vi "test malformed json.vi"(8 "error in (no error)":errorcluster) -> (0 "error out":errorcluster, 3 "body":string)   [LabVIEW 2020, in "MCP Server tests.lvlib"]
doc: "A body that is not valid JSON cannot be read: JSON-RPC error -32700 (Parse error) with id null, even if the text contains something that looks like an id."
uses:
  MCP Server tests.lvlib
  <vilib>/JDP Science/JSONtext/Next JSON Value.vi
  <vilib>/JDP Science/JSONtext/String Subset.vi
  <vilib>/JDP Science/JSONtext/Parsing/Advance past next JSON Value (inlined COPY).vi
  <vilib>/JDP Science/JSONtext/Parsing/Advance past whitespace.vi
  <vilib>/JDP Science/JSONtext/Parsing/Advance past String.vi
  <vilib>/JDP Science/JSONtext/Parsing/Advance past Number.vi
  <vilib>/JDP Science/JSONtext/Parsing/Advance past Line Ending.vi
  <vilib>/JDP Science/JSONtext/Parsing/Parse Full Path or Item Name.vi
  <vilib>/JDP Science/JSONtext/Parsing/Advance past Array.vi
  <vilib>/JDP Science/JSONtext/Parsing/Advance past Object.vi
  <vilib>/JDP Science/JSONtext/support/Error Cluster From Code.vi
  <vilib>/JDP Science/JSONtext/Offset/Find Item Locations by Path.vi
  <vilib>/addons/_JKI Toolkits/Caraya/classes/Test/Test.lvclass
  <vilib>/JDP Science/JSONtext/JSONtext.lvlib
  <vilib>/addons/_JKI Toolkits/Caraya/classes/Assert/Assert.lvclass
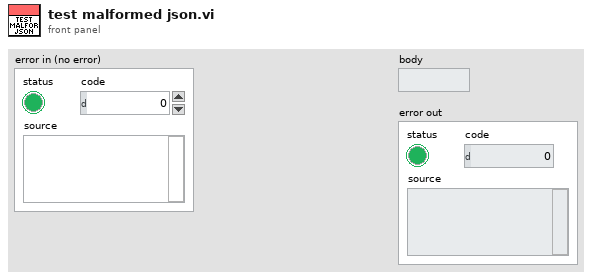
[diagram p1: front panel]
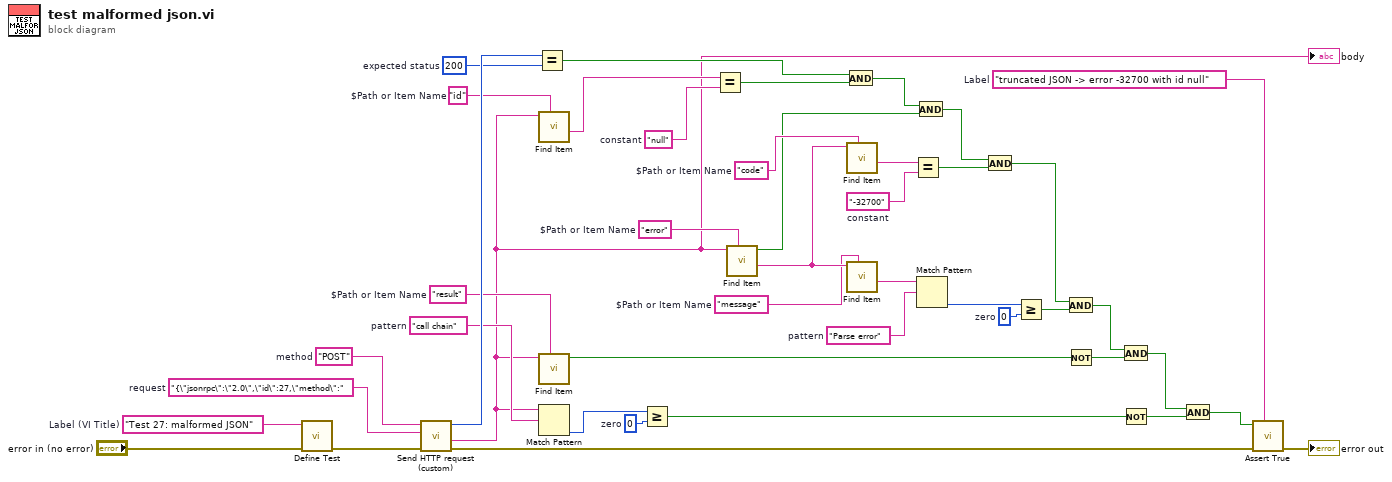
[diagram p0: block diagram]
diagram:
  w3 = "truncated JSON -> error -32700 with id null"  # Label
  w19 = 0  # zero
  w21 = "call chain"  # pattern
  w23 = 0  # zero
  w25 = "Parse error"  # pattern
  w27 = "-32700"  # constant
  w29 = "null"  # constant
  w31 = "result"  # $Path or Item Name
  w32 = "message"  # $Path or Item Name
  w34 = "code"  # $Path or Item Name
  w35 = "error"  # $Path or Item Name
  w36 = "id"  # $Path or Item Name
  w37 = 200  # expected status
  w40 = "{\"jsonrpc\":\"2.0\",\"id\":27,\"method\":"  # request
  w41 = "POST"  # method
  w43 = "Test 27: malformed JSON"  # Label (VI Title)
  n1 = call <vilib>:"Define Test.vi"("error in (no error)"="error in (no error)", "Label (VI Title)"=w43) -> ("error out"=w39:errorcluster)  [unwired: 8 in, 1 out]
  n2 = call "Send HTTP request (custom).vi"("error in (no error)"=w39, "request"=w40, "method"=w41) -> ("error out"=w4:errorcluster, "response"=w2:string, "status code"=w38:i32)  [unwired: 5 in, 1 out]
  "body" <- w2
  n3 = Equal?(x=w38, y=w37) -> (x = y?=w17:bool)
  n4 = call <vilib>:"Find Item.vi"("$Path or Item Name"=w36, "JSON"=w2) -> ("<JSON>"=w30:string)  [unwired: 6 in, 3 out]
  n5 = call <vilib>:"Find Item.vi"("$Path or Item Name"=w31, "JSON"=w2) -> ("Found"=w22:bool)  [unwired: 6 in, 3 out]
  n6 = Match Pattern(string=w2, regular expression=w21) -> (offset past match=w20:i32)  [unwired: 1 in, 3 out]
  n7 = Greater Or Equal?(x=w20, y=w19) -> (x >= y?=w18:bool)
  n8 = Equal?(x=w30, y=w29) -> (x = y?=w16:bool)
  n9 = call <vilib>:"Find Item.vi"("$Path or Item Name"=w35, "JSON"=w2) -> ("<JSON>"=w33:string, "Found"=w14:bool)  [unwired: 6 in, 2 out]
  n10 = And(x=w17, y=w16) -> (x .and. y?=w15:bool)
  n11 = call <vilib>:"Find Item.vi"("$Path or Item Name"=w34, "JSON"=w33) -> ("<JSON>"=w28:string)  [unwired: 6 in, 3 out]
  n12 = call <vilib>:"Find Item.vi"("$Path or Item Name"=w32, "JSON"=w33) -> ("<JSON>"=w26:string)  [unwired: 6 in, 3 out]
  n13 = Equal?(x=w28, y=w27) -> (x = y?=w12:bool)
  n14 = And(x=w15, y=w14) -> (x .and. y?=w13:bool)
  n15 = Match Pattern(string=w26, regular expression=w25) -> (offset past match=w24:i32)  [unwired: 1 in, 3 out]
  n16 = And(x=w13, y=w12) -> (x .and. y?=w11:bool)
  n17 = Greater Or Equal?(x=w24, y=w23) -> (x >= y?=w10:bool)
  n18 = And(x=w11, y=w10) -> (x .and. y?=w9:bool)
  n19 = Not(x=w22) -> (.not. x?=w8:bool)
  n20 = And(x=w9, y=w8) -> (x .and. y?=w7:bool)
  n21 = Not(x=w18) -> (.not. x?=w6:bool)
  n22 = And(x=w7, y=w6) -> (x .and. y?=w5:bool)
  n23 = call <vilib>:"Assert True.vi"("Label"=w3, "error in (no error)"=w4, "True?"=w5) -> ("error out"=→"error out":errorcluster)  [unwired: 7 in, 1 out]
